vi "append_console_string.vi"(8 "error in (no error)":errorcluster, 9 "color":u32(colorbox), 10 "newline":string, 11 "console (in)":refnum<vi>) -> (0 "error out":errorcluster, 3 "reference out":refnum<vi>)   [LabVIEW 2021, in "console.provider.lvclass"]
uses:
  console.provider.lvclass
  console.provider.lvclass/console.provider.ctl
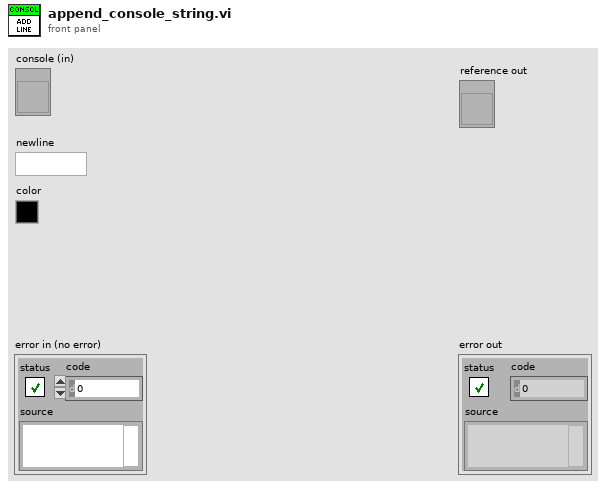
[diagram p1: front panel]
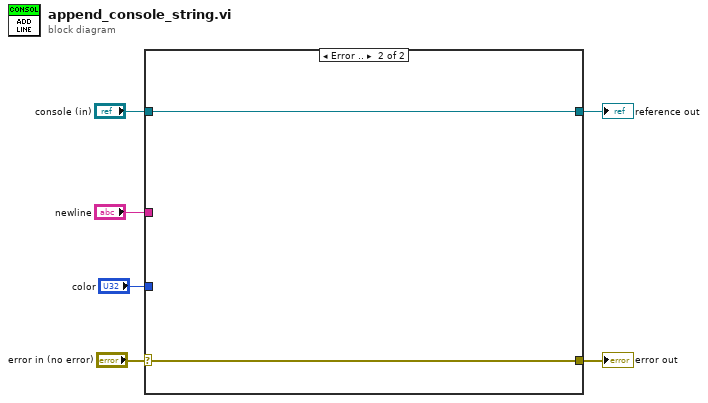
[diagram p0: block diagram]
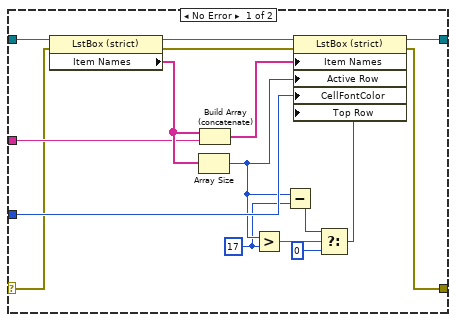
[diagram p2: hidden frame]
diagram:
  n1 = case shown="Error .." "error in (no error)" {
    selector: "error in (no error)" -> [w7 w23]
    tunnel: "console (in)" -> [w22 w24]
    tunnel: "newline" -> [w20 _]
    tunnel: "color" -> [w17 _]
    tunnel: [w16 w23] -> w3
    tunnel: [w14 w24] -> w2
    frame No Error {
      w11 = 17 ("y")
      n2 = property class="LstBox (strict)"(reference=w22, error in=w7) -> (reference out=w19:refnum<vi>, error out=w15:errorcluster, "Item Names"=w21:string[])
      n3 = Array Size(array=w21) -> (size(s)=w12:i32)
      n4 = Build Array (concatenate)(w21, w20) -> (w18:string[])
      n5 = Greater?(x=w12, y=w11) -> (0:w13:bool)
      n6 = Subtract(x=w12, y=w11) -> (x-y=w10:i32)
      n7 = Select(t=w10, s=w13, f=0) -> (s? t:f=w8:i32)
      n8 = property class="LstBox (strict)"(reference=w19, error in=w15, "Item Names"=w18, "Active Row"=w12, "CellFontColor"=w17, "Top Row"=w8) -> (reference out=w14:refnum<vi>, error out=w16:errorcluster)
    }
    frame Error {
    }
  }
  "error out" <- w3
  "reference out" <- w2
